vi "AlliGator Dock-Undock Subpanel Event.vi"(8 "Error In":errorcluster, 10 "Dock?":bool, 11 "VI in":refnum<vi>) -> (0 "Error Out":errorcluster)   [LabVIEW 2021, in "AlliGator GUI.lvlib"]
uses:
  AlliGator GUI.lvlib
  AlliGator Subpanel Event Data.ctl
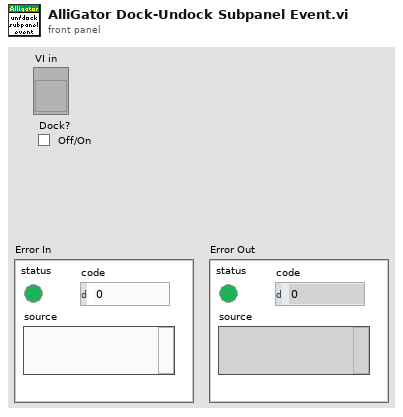
[diagram p1: front panel]
types:
  T1 = typedef "AlliGator GUI.lvlib/AlliGator Subpanel Event Data.ctl" = cluster{"subpanel":string, "event":string}
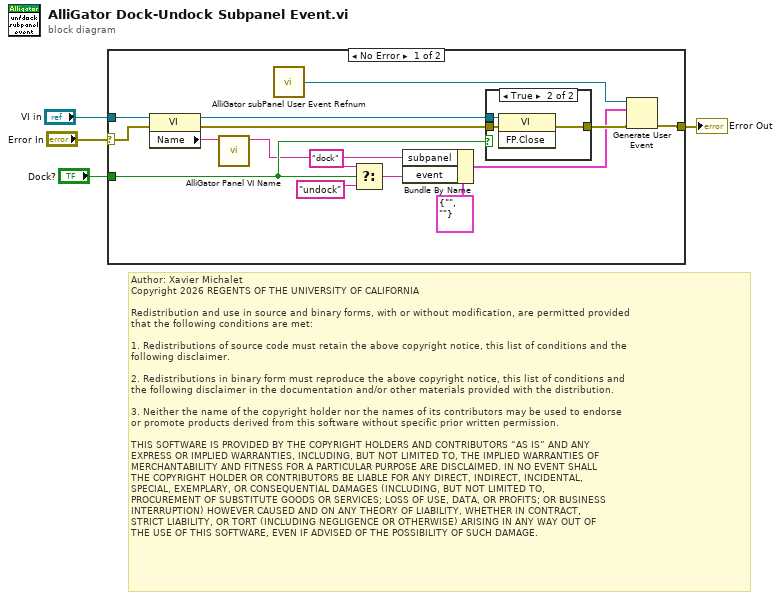
[diagram p0: block diagram]
diagram:
  # "Author: Xavier Michalet\nCopyright 2026 REGENTS OF THE UNIVERSITY OF CALIFORNIA\n\nRedistribution and use in source and binary forms, with or without modification, are permitted provided\nthat the following conditions are met:\n\n1. Redistributions of source code must retain the above copyright notice, this list of conditions and the\nfollowing disclaimer.\n\n2. Redistributions in binary form must reproduce the above copyright notice, this list of conditions and\nthe following disclaimer in the documentation and/or other materials provided with the distribution.\n\n3. Neither the name of the copyright holder nor the names of its contributors may be used to endorse \nor promote products derived from this software without specific prior written permission.\n\nTHIS SOFTWARE IS PROVIDED BY THE COPYRIGHT HOLDERS AND CONTRIBUTORS “AS IS” AND ANY \nEXPRESS OR IMPLIED WARRANTIES, INCLUDING, BUT NOT LIMITED TO, THE IMPLIED WARRANTIES OF\nMERCHANTABILITY AND FITNESS FOR A PARTICULAR PURPOSE ARE DISCLAIMED. IN NO EVENT SHALL\nTHE COPYRIGHT HOLDER OR CONTRIBUTORS BE LIABLE FOR ANY DIRECT, INDIRECT, INCIDENTAL, \nSPECIAL, EXEMPLARY, OR CONSEQUENTIAL DAMAGES (INCLUDING, BUT NOT LIMITED TO, \nPROCUREMENT OF SUBSTITUTE GOODS OR SERVICES; LOSS OF USE, DATA, OR PROFITS; OR BUSINESS\nINTERRUPTION) HOWEVER CAUSED AND ON ANY THEORY OF LIABILITY, WHETHER IN CONTRACT, \nSTRICT LIABILITY, OR TORT (INCLUDING NEGLIGENCE OR OTHERWISE) ARISING IN ANY WAY OUT OF\nTHE USE OF THIS SOFTWARE, EVEN IF ADVISED OF THE POSSIBILITY OF SUCH DAMAGE."
  n1 = case shown="No Error" "Error In" {
    selector: "Error In" -> [w14 w24]
    tunnel: "VI in" -> [w18 _]
    tunnel: "Dock?" -> [w11 _]
    tunnel: [w7 w24] -> w1
    frame No Error {
      n2 = property class="VI"(reference=w18, error in=w14) -> (reference out=w13:refnum<vi>, error out=w12:errorcluster, "Name"=w5:string)
      n3 = call "AlliGator Panel VI Name.vi"("Panel VI Name"=w5) -> ("Panel Name"=w6:string)  [unwired: 10 in]
      n4 = call "AlliGator subPanel User Event Refnum.vi"() -> ("subPanel Event"=w8:refnum<user-event>)  [unwired: 9 in]
      n5 = Select(t="dock" ("event"), s=w11, f="undock") -> (s? t:f=w16:string)
      n6 = Bundle By Name(cluster=T1 {"subpanel"="", "event"=""} ("Subpanel Event"), "subpanel"=w6, "event"=w16) -> (w9:T1)
      n7 = case shown="True" w11 {
        tunnel: [w20 w23] -> w10
        tunnel: w13 -> [_ w22]
        tunnel: w12 -> [w20 w21]
        frame False {
        }
        frame True {
          n8 = invoke class="VI" method="FP.Close"(reference=w22, error in=w21) -> (error out=w23:errorcluster)  [unwired: 1 in, 2 out]
        }
      }
      n9 = Generate User Event(user event=w8, event data cluster=w9, error in=w10) -> (error out=w7:errorcluster)  [unwired: 1 in, 1 out]
    }
    frame Error {
    }
  }
  "Error Out" <- w1
